vi "pwmSetRange.vi"(8 "error in (no error)":errorcluster, 10 "Value":i32, 11 "RPi Pin":T1) -> (0 "error out":errorcluster, 3 "RPi Pin out":T1)   [LabVIEW 2020, in "wiringPi.lvlib"]
doc: "<b>_______________________________________________________________</b>\n** Author: Juan José Villacorta\n** LabVIEW wrapper for C library <b> wiringPi </b>,\n** https://github.com/WiringPi/WiringPi\n<b>_______________________________________________________________</b>\n\n/*\n * pwmSetRange:\n * Set the PWM range register. We set both range registers to the same\n * value. If you want different in your own code, then write your own.\n *********************************************************************************\n */"
uses:
  wiringPi.lvlib
  Type Defs/GPIO Pins.ctl
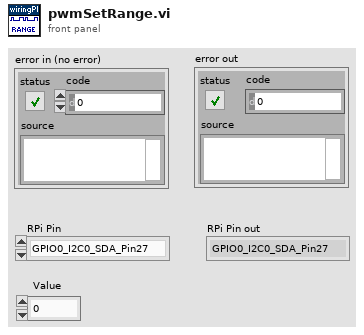
[diagram p1: front panel]
types:
  T1 = typedef "wiringPi.lvlib/GPIO Pins.ctl" = enum32{"GPIO0_I2C0_SDA_Pin27", "GPIO1_I2C0_SDA1_Pin28", "GPIO2_I2C1_SDA_Pin3", "GPIO3_I2C1_SCL_Pin5", "GPIO4_GPCLK0_Pin7", "GPIO5_GPCLK1_Pin29", "GPIO6_GPCLK2_Pin31", "GPIO7_SPI_CE1_N_Pin26", "GPIO8_SPI_CE0_N_Pin24", "GPIO9_SPI0_MISO_Pin21", "GPIO10_SPI0_MOSI_Pin19", "GPIO11_SPI0_CLK_Pin23", "GPIO12_PWM0_Pin32", "GPIO13_PWM1_Pin33", "GPIO14_TXD0_Pin8", "GPIO15_RXD0_Pin10", "GPIO16_Pin36", "GPIO17_Pin11", "GPIO18_PWM0_Pin12", "GPIO19_PWM1_Pin35", "GPIO20_GPCLK0_Pin38", "GPIO21_GPCLK1_Pin40", "GPIO22_Pin15", "GPIO23_Pin16", "GPIO24_Pin18", "GPIO25_Pin22", "GPIO26_Pin37", "GPIO27_Pin13"}
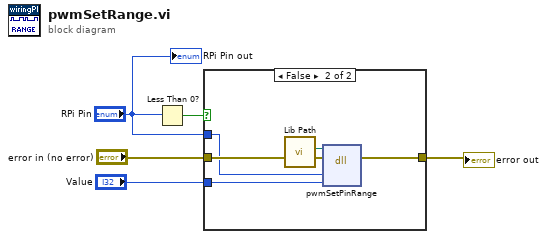
[diagram p0: block diagram]
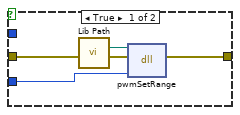
[diagram p2: hidden frame]
diagram:
  n1 = Less Than 0?(x="RPi Pin") -> (x < 0?=w2:bool)
  n2 = case shown="False" w2 {
    tunnel: "error in (no error)" -> [w9 w14]
    tunnel: [w8 w13] -> w4
    tunnel: "Value" -> [w7 w12]
    tunnel: "RPi Pin" -> [_ w10]
    frame True {
      n3 = call "Lib Path.vi"() -> ("path out"=w6:path)  [unwired: 11 in]
      n4 = dll-call lib="libLVwiringPI.so" fn="pwmSetRange"(path in=w6, error in=w9, "value"=w7) -> (error out=w8:errorcluster)  [unwired: 3 in, 1 out]
    }
    frame False {
      n5 = call "Lib Path.vi"() -> ("path out"=w11:path)  [unwired: 11 in]
      n6 = dll-call lib="libLVwiringPI.so" fn="pwmSetPinRange"(path in=w11, error in=w14, "pin"=w10, "value"=w12) -> (error out=w13:errorcluster)  [unwired: 4 in, 1 out]
    }
  }
  "error out" <- w4
  "RPi Pin out" <- "RPi Pin"
